vi "GOOP300_FindFilesToExchange.vi"(0 "OldClassName(Prefix or suffix for some VIs)":string="NotUsedIfNotWired", 1 "OldFolderPath":path, 2 "NewFolderPath":path, 3 "NewClassName(Prefix or suffix for some VIs)":string="NotUsedIfNotWired") -> (15 "OldFiles":path[](array[path]), 16 "NewFileArray":path[](array[path]))   [LabVIEW 2020]
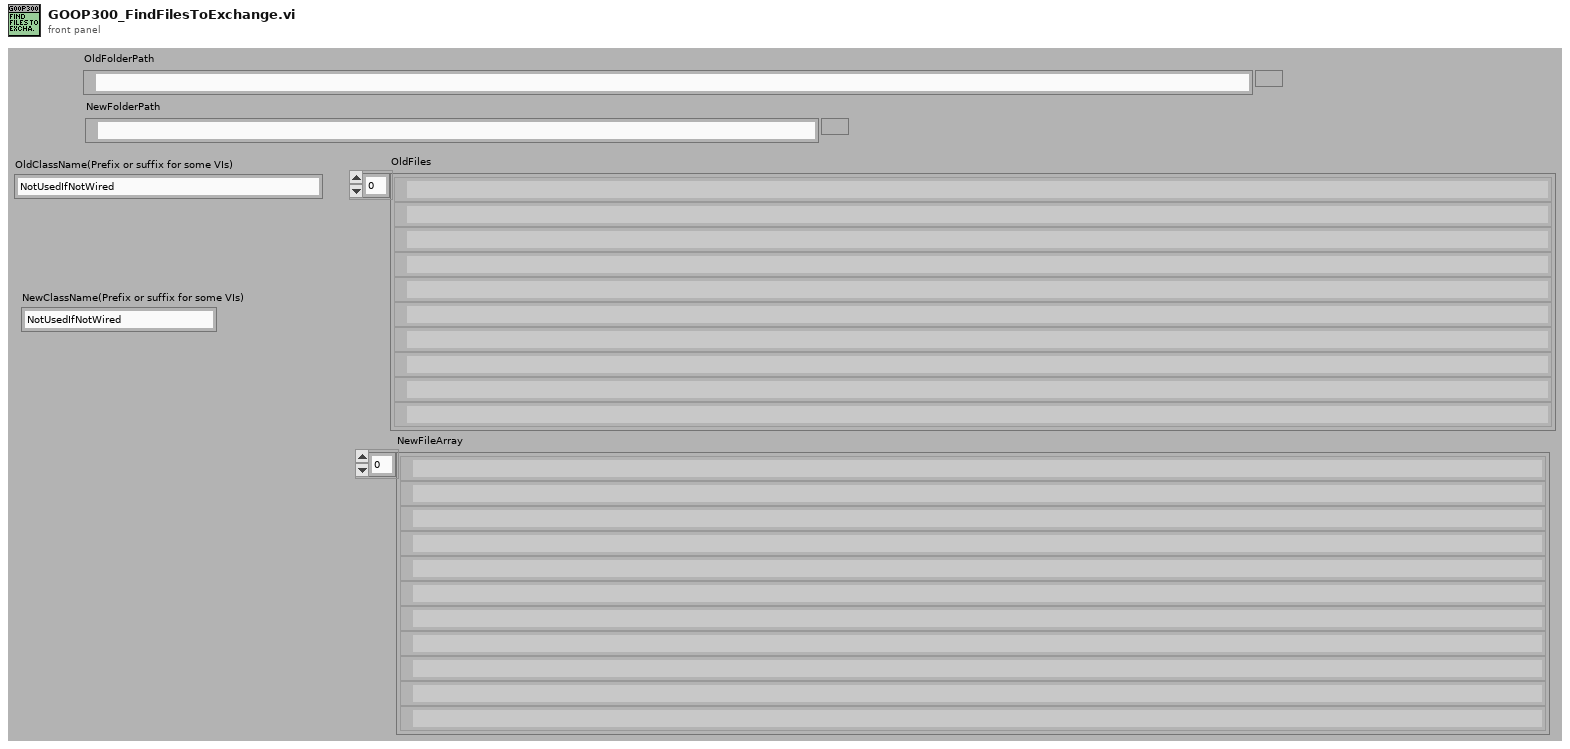
[diagram p1: front panel]
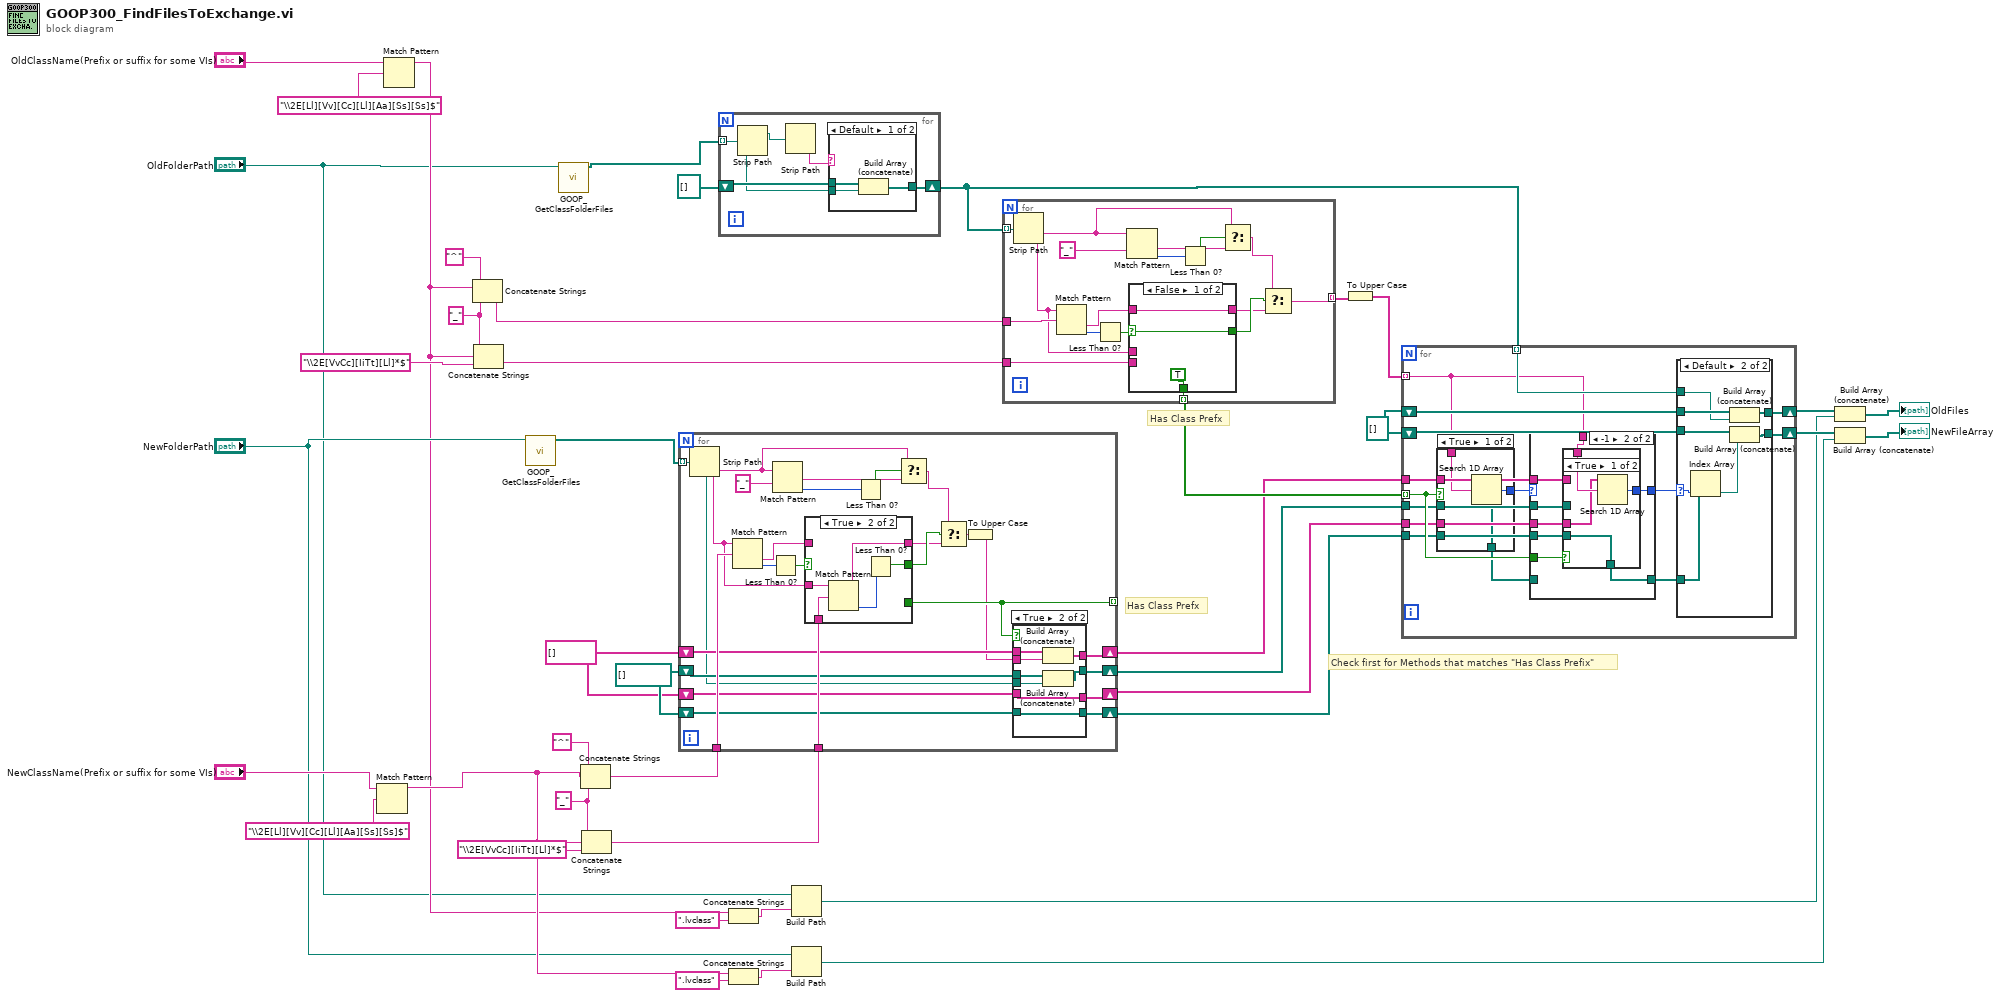
[diagram p0: block diagram]
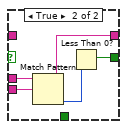
[diagram p2: hidden frame]
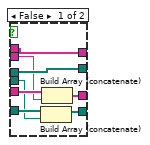
[diagram p3: hidden frame]
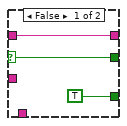
[diagram p4: hidden frame]
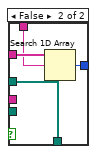
[diagram p6: hidden frame]
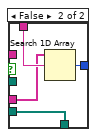
[diagram p7: hidden frame]
diagram:
  w23 = path[] []
  w22 = string[] []
  w26 = "_" ("regular expression")
  w37 = "_" ("regular expression")
  w40 = path[] []
  # "Check first for Methods that matches \"Has Class Prefix\""
  # "Has Class Prefx"
  # "Has Class Prefx"
  n1 = Match Pattern(string="NewClassName(Prefix or suffix for some VIs)", regular expression="\\2E[Ll][Vv][Cc][Ll][Aa][Ss][Ss]$") -> (before substring=w10:string)  [unwired: 1 in, 3 out]
  n2 = Match Pattern(string="OldClassName(Prefix or suffix for some VIs)", regular expression="\\2E[Ll][Vv][Cc][Ll][Aa][Ss][Ss]$") -> (before substring=w4:string)  [unwired: 1 in, 3 out]
  n3 = Concatenate Strings("^" ("string"), w4, w26) -> (w25:string)
  n4 = Concatenate Strings(w26, w4, "\\2E[VvCc][IiTt][Ll]*$" ("string")) -> (w24:string)
  n5 = call "GOOP_GetClassFolderFiles.vi"("NewFolderPath"="NewFolderPath") -> ("Array"=w16:path[])  [unwired: 10 in]
  n6 = call "GOOP_GetClassFolderFiles.vi"("NewFolderPath"="OldFolderPath") -> ("Array"=w13:path[])  [unwired: 10 in]
  n7 = Concatenate Strings("^" ("string"), w10, w37) -> (w38:string)
  n8 = Concatenate Strings(w37, w10, "\\2E[VvCc][IiTt][Ll]*$" ("string")) -> (w34:string)
  n9 = for {
    tunnel: w16 -> [w51] mode=indexing
    tunnel: w38 -> [w64]
    tunnel: w34 -> [w57]
    tunnel: [w49] -> _ mode=indexing
    shift-right: [w53] -> w18
    shift-left: w22 -> [w54]
    shift-right: [w50] -> w17
    shift-left: w23 -> [w52]
    shift-right: [w47] -> w15
    shift-left: w22 -> [w46]
    shift-right: [w48] -> w14
    shift-left: w23 -> [w45]
    n10 = Strip Path(path=w51) -> (name=w55:string)  [unwired: 1 out]
    n11 = Match Pattern(string=w55, regular expression=w64) -> (after substring=w59:string, offset past match=w63:i32)  [unwired: 1 in, 2 out]
    n12 = Less Than 0?(x=w63) -> (x < 0?=w61:bool)
    n13 = Match Pattern(string=w55, regular expression="_") -> (after substring=w56:string, offset past match=w67:i32)  [unwired: 1 in, 2 out]
    n14 = case shown="True" w61 {
      selector: w61 -> [w86 _]
      tunnel: [w86 w91] -> w60
      tunnel: w59 -> [w85 _]
      tunnel: [w85 w90] -> w58
      tunnel: w55 -> [_ w88]
      tunnel: w57 -> [_ w87]
      tunnel: [TRUE _] -> w49
      frame False {
      }
      frame True {
        n15 = Match Pattern(string=w88, regular expression=w87) -> (before substring=w90:string, offset past match=w89:i32)  [unwired: 1 in, 2 out]
        n16 = Less Than 0?(x=w89) -> (x < 0?=w91:bool)
      }
    }
    n17 = Less Than 0?(x=w67) -> (x < 0?=w66:bool)
    n18 = Select(t=w55, s=w66, f=w56) -> (s? t:f=w62:string)
    n19 = Select(t=w62, s=w60, f=w58) -> (s? t:f=w44:string)
    n20 = To Upper Case(1:w44) -> (0:w43:string)
    n21 = case shown="True" w49 {
      tunnel: w54 -> [w75 w83]
      tunnel: w43 -> [w69 w82]
      tunnel: [w75 w81] -> w53
      tunnel: w52 -> [w74 w80]
      tunnel: w51 -> [w68 w79]
      tunnel: [w74 w78] -> w50
      tunnel: [w73 w77] -> w47
      tunnel: [w72 w76] -> w48
      tunnel: w46 -> [w71 w77]
      tunnel: w45 -> [w70 w76]
      frame False {
        n22 = Build Array (concatenate)(w70, w68) -> (w72:path[])
        n23 = Build Array (concatenate)(w71, w69) -> (w73:string[])
      }
      frame True {
        n24 = Build Array (concatenate)(w83, w82) -> (w81:string[])
        n25 = Build Array (concatenate)(w80, w79) -> (w78:path[])
      }
    }
  }
  n26 = for {
    tunnel: w13 -> [w92] mode=indexing
    shift-right: [w93] -> w29
    shift-left: path[] [] -> [w94]
    n27 = Strip Path(path=w92) -> (stripped path=w96:path)  [unwired: 1 out]
    n28 = Strip Path(path=w96) -> (name=w95:string)  [unwired: 1 out]
    n29 = case shown="Default" w95 {
      tunnel: w94 -> [w99 w100]
      tunnel: [w98 w100] -> w93
      tunnel: w92 -> [w97 _]
      frame Default {
        n30 = Build Array (concatenate)(w99, w97) -> (w98:path[])
      }
      frame "Methods" {
      }
    }
  }
  n31 = Concatenate Strings(w4, ".lvclass" ("string")) -> (w6:string)
  n32 = Concatenate Strings(w10, ".lvclass" ("string")) -> (w8:string)
  n33 = Build Path(base path="OldFolderPath", name or relative path=w6) -> (appended path=w2:path)
  n34 = Build Path(base path="NewFolderPath", name or relative path=w8) -> (appended path=w1:path)
  n35 = for {
    tunnel: w29 -> [w116] mode=indexing
    tunnel: [w109] -> w21 mode=indexing
    tunnel: w25 -> [w104]
    tunnel: w24 -> [w103]
    tunnel: [w101] -> w19 mode=indexing
    n36 = Strip Path(path=w116) -> (name=w102:string)  [unwired: 1 out]
    n37 = Match Pattern(string=w102, regular expression=w104) -> (after substring=w106:string, offset past match=w111:i32)  [unwired: 1 in, 2 out]
    n38 = Less Than 0?(x=w111) -> (x < 0?=w108:bool)
    n39 = Match Pattern(string=w102, regular expression="_") -> (after substring=w114:string, offset past match=w115:i32)  [unwired: 1 in, 2 out]
    n40 = case shown="False" w108 {
      selector: w108 -> [w119 _]
      tunnel: [w119 w124] -> w107
      tunnel: w106 -> [w118 _]
      tunnel: [w118 w123] -> w105
      tunnel: w102 -> [_ w121]
      tunnel: w103 -> [_ w120]
      tunnel: [TRUE _] -> w101
      frame False {
      }
      frame True {
        n41 = Match Pattern(string=w121, regular expression=w120) -> (before substring=w123:string, offset past match=w122:i32)  [unwired: 1 in, 2 out]
        n42 = Less Than 0?(x=w122) -> (x < 0?=w124:bool)
      }
    }
    n43 = Less Than 0?(x=w115) -> (x < 0?=w113:bool)
    n44 = Select(t=w102, s=w113, f=w114) -> (s? t:f=w110:string)
    n45 = Select(t=w110, s=w107, f=w105) -> (s? t:f=w109:string)
  }
  n46 = To Upper Case(1:w21) -> (0:w20:string[])
  n47 = for {
    tunnel: w20 -> [w128] mode=indexing
    tunnel: w18 -> [w129]
    tunnel: w29 -> [w139] mode=indexing
    shift-right: [w137] -> w41
    shift-left: w40 -> [w138]
    shift-right: [w136] -> w42
    shift-left: w40 -> [w135]
    tunnel: w17 -> [w130]
    tunnel: w19 -> [w133] mode=indexing
    tunnel: w15 -> [w132]
    tunnel: w14 -> [w131]
    n48 = case shown="True" w133 {
      tunnel: w129 -> [w161 _]
      tunnel: [w160 w165] -> w134
      tunnel: w128 -> [w159 w164]
      tunnel: w130 -> [w158 _]
      tunnel: w132 -> [_ w163]
      tunnel: w131 -> [_ w162]
      tunnel: [w158 w162] -> w127
      frame True {
        n49 = Search 1D Array(1D array=w161, element=w159) -> (index of element=w160:i32)  [unwired: 1 in]
      }
      frame False {
        n50 = Search 1D Array(1D array=w163, element=w164) -> (index of element=w165:i32)  [unwired: 1 in]
      }
    }
    n51 = case shown="-1" w134 {
      selector: w134 -> [w140 _]
      tunnel: w133 -> [_ w149]
      tunnel: w132 -> [_ w148]
      tunnel: w131 -> [_ w147]
      tunnel: w130 -> [_ w146]
      tunnel: w129 -> [_ w145]
      tunnel: w128 -> [_ w144]
      tunnel: w127 -> [w141 _]
      tunnel: [w141 w142] -> w126
      tunnel: [w140 w143] -> w125
      frame 0, Default {
      }
      frame -1 {
        n52 = case shown="True" w149 {
          tunnel: w145 -> [_ w157]
          tunnel: [w153 w156] -> w143
          tunnel: w144 -> [w152 w155]
          tunnel: w146 -> [_ w154]
          tunnel: w148 -> [w151 _]
          tunnel: w147 -> [w150 _]
          tunnel: [w150 w154] -> w142
          frame True {
            n53 = Search 1D Array(1D array=w151, element=w152) -> (index of element=w153:i32)  [unwired: 1 in]
          }
          frame False {
            n54 = Search 1D Array(1D array=w157, element=w155) -> (index of element=w156:i32)  [unwired: 1 in]
          }
        }
      }
    }
    n55 = case shown="Default" w125 {
      selector: w125 -> [_ w170]
      tunnel: w139 -> [_ w174]
      tunnel: w138 -> [w166 w175]
      tunnel: [w166 w173] -> w137
      tunnel: [w167 w172] -> w136
      tunnel: w135 -> [w167 w171]
      tunnel: w126 -> [_ w168]
      frame -1 {
      }
      frame Default {
        n56 = Index Array(array=w168, index=w170) -> (element=w169:path)
        n57 = Build Array (concatenate)(w175, w174) -> (w173:path[])
        n58 = Build Array (concatenate)(w171, w169) -> (w172:path[])
      }
    }
  }
  n59 = Build Array (concatenate)(w41, w2) -> (→"OldFiles":path[])
  n60 = Build Array (concatenate)(w42, w1) -> (→"NewFileArray":path[])
